vi "DVR Get File Config.vi"(8 "error in (no error)":errorcluster) -> (0 "error out":errorcluster, 3 "Config":T1)   [LabVIEW 2019, in "Language Selection.lvlib"]
doc: "Converts the Data Value Reference back into Controls translation.\n- - -\nCopyright (c) 2026, Merecs Engineering GmbH"
uses:
  Language Selection.lvlib
  TypeDefs/Cluster Language Configuration.ctl
  community/Cluster Settings Data.ctl
  TypeDefs/Cluster Language.ctl
  TypeDefs/Cluster PropertyTranslation.ctl
  TypeDefs/Enum Property Type.ctl
  Global Language Selection.vi
panel:
  # "Connector Pane"
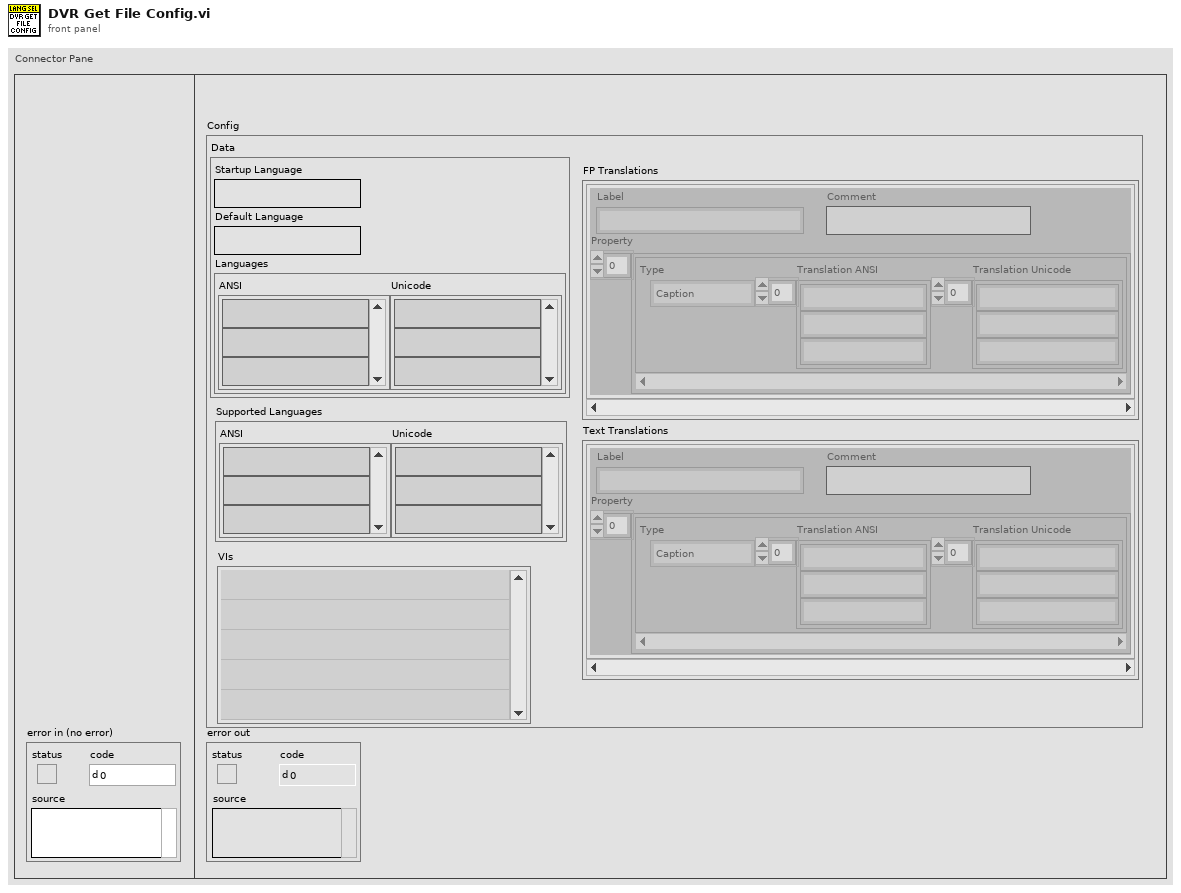
[diagram p1: front panel]
types:
  T1 = typedef "Language Selection.lvlib/Cluster Language Configuration.ctl" = cluster{"Data":T2, "Supported Languages":cluster{"ANSI":string[], "Unicode":string[]}, "VIs":path[], "FP Translations":T3[], "Text Translations":T3[]}
  T2 = typedef "Language Selection.lvlib/Cluster Settings Data.ctl" = cluster{"Startup Language":string, "Default Language":string, "Languages":cluster{"ANSI":string[], "Unicode":string[]}}
  T3 = typedef "Language Selection.lvlib/Cluster Language.ctl" = cluster{"Label":string, "Comment":string, "Property":T4[]}
  T4 = typedef "Language Selection.lvlib/Cluster PropertyTranslation.ctl" = cluster{"Type":T5, "Translation ANSI":string[], "Translation Unicode":string[]}
  T5 = typedef "Language Selection.lvlib/Enum Property Type.ctl" = enum16{"NA", "Caption", "String Value", "Boolean Text", "Ring Strings", "1D Array Elements", "2D Array Elements", "(MC)Listbox Header", "(MC)Listbox Items", "Tab Pages Names", "X & Y GraphChart", "Plot Names", "Table Headers", "Table Items", "TipStrip", "Combobox Strings", "Cursor Name", "Tree Col Headers"}
  T6 = typedef "Language Selection.lvlib/Cluster DVR.ctl" = cluster{"Data":T2, "VIs":path[], "FP Translation":map{string, T7}, "Text Translation":map{string, T7}, "Front panels":set{refnum<vi>}}
  T7 = typedef "Language Selection.lvlib/Cluster LanguageClusterWithRefnum.ctl" = cluster{"Property":T4[], "Controls":set{refnum<vi>}}
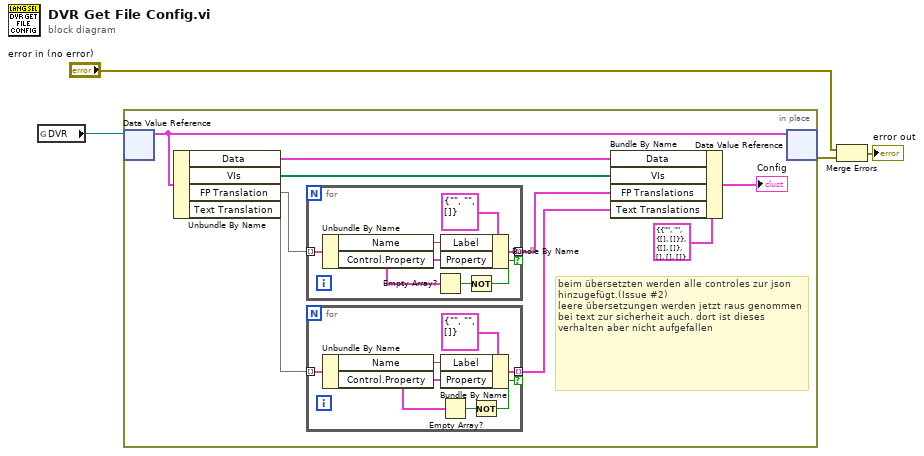
[diagram p0: block diagram]
diagram:
  n1 = global read "Global Language Selection.vi" "DVR"() -> (w1:refnum<data-value>)
  n2 = in-place "In Place Element Structure" {
    # "beim übersetzten werden alle controles zur json hinzugefügt.(Issue #2)\nleere übersetzungen werden jetzt raus genommen \nbei text zur sicherheit auch. dort ist dieses verhalten aber nicht aufgefallen"
    n3 = in-place-dvr #1(w1) -> (w13:T6)  [unwired: 1 out]
    n4 = Unbundle By Name(w13) -> ("Data"=w11:T2, "VIs"=w10:path[], "FP Translation"=w9:map{string, T7}, "Text Translation"=w6:map{string, T7})
    n5 = for {
      tunnel: w9 -> [w26] mode=indexing
      tunnel: [w24] -> w7 mode=indexing if=w21
      n6 = Unbundle By Name(w26) -> ("Name"=w25:string, "Control.Property"=w23:T4[])
      n7 = Empty Array?(array=w23) -> (empty?=w22:bool)
      n8 = Bundle By Name(cluster=T3 {"Label"="", "Comment"="", "Property"=[]} ("Control"), "Label"=w25, "Property"=w23) -> (w24:T3)
      n9 = Not(x=w22) -> (.not. x?=w21:bool)
    }
    n10 = for {
      tunnel: w6 -> [w19] mode=indexing
      tunnel: [w17] -> w5 mode=indexing if=w14
      n11 = Unbundle By Name(w19) -> ("Name"=w18:string, "Control.Property"=w15:T4[])
      n12 = Empty Array?(array=w15) -> (empty?=w16:bool)
      n13 = Bundle By Name(cluster=T3 {"Label"="", "Comment"="", "Property"=[]} ("Control"), "Label"=w18, "Property"=w15) -> (w17:T3)
      n14 = Not(x=w16) -> (.not. x?=w14:bool)
    }
    n15 = Bundle By Name(cluster=T1 {"Data"={"Startup Language"="", "Default Language"="", "Languages"={"ANSI"=[], "Unicode"=[]}}, "Supported Languages"={"ANSI"=[], "Unicode"=[]}, "VIs"=[], "FP Translations"=[], "Text Translations"=[]} ("Langúage Selection"), "Data"=w11, "VIs"=w10, "FP Translations"=w7, "Text Translations"=w5) -> (→"Config":T1)
    n16 = in-place-dvr #1(w13) -> (w3:errorcluster)  [unwired: 1 out]
  }
  n17 = Merge Errors("error in (no error)", w3) -> (→"error out":errorcluster)
